vi "Advance Stories.vi"(11 "market":T1) -> (3 "market out":T1)   [LabVIEW 2020, in "Full Featured MCP Server.lvlib"]
doc: "Publishes the story steps that are due. After a step the story takes its good or its bad branch (Good Outcome.vi with the odds of the step and the quality of the lead stock) and the next step is scheduled; a story without a next step ends. Stories that are not due yet wait."
uses:
  Full Featured MCP Server.lvlib
  Market State.ctl
  News Item.ctl
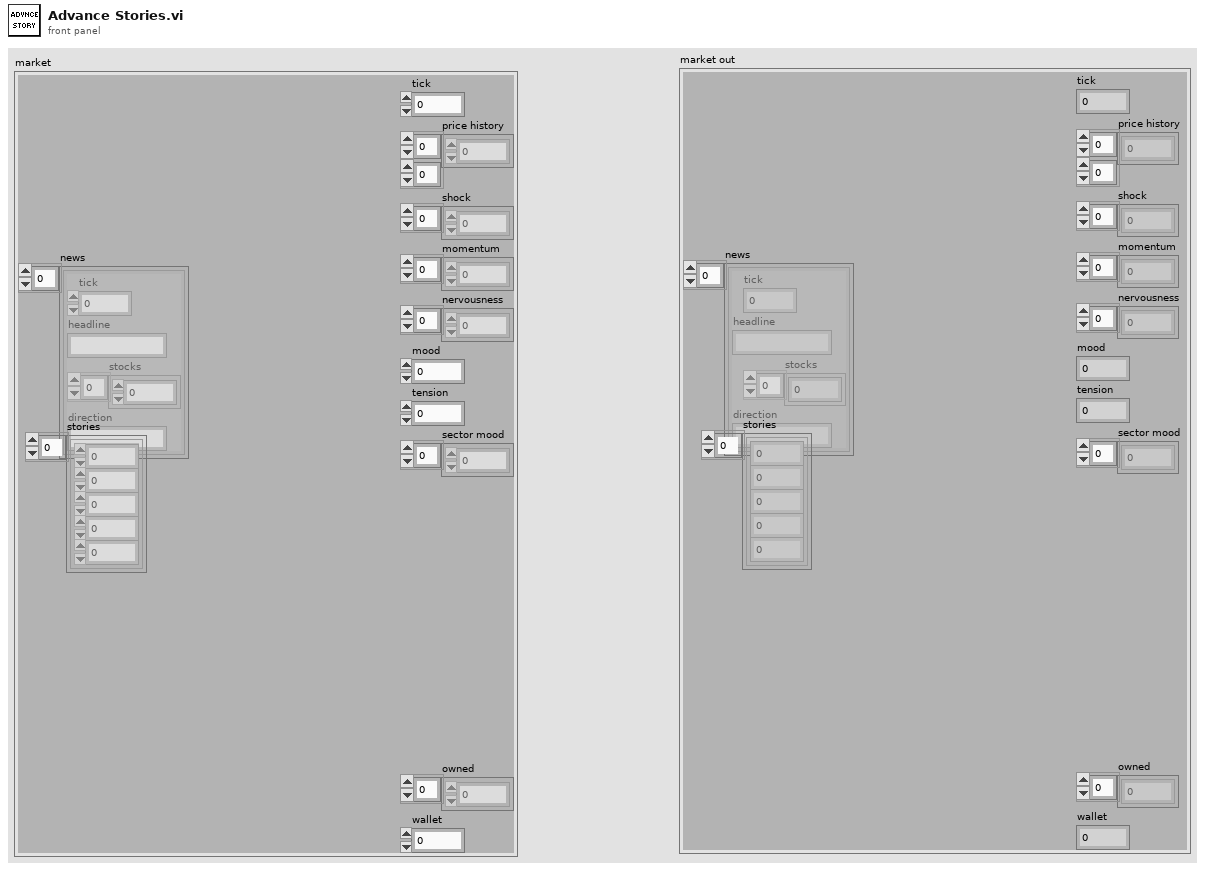
[diagram p1: front panel]
types:
  T1 = typedef "Full Featured MCP Server.lvlib/Market State.ctl" = cluster{"tick":i32, "price history":dbl[][], "shock":dbl[], "momentum":dbl[], "nervousness":dbl[], "mood":dbl, "tension":dbl, "sector mood":dbl[], "news":T2[], "stories":cluster{"arc":i32, "step":i32, "due":i32, "stock":i32, "other":i32}[], "owned":i32[], "wallet":dbl}
  T2 = typedef "Full Featured MCP Server.lvlib/News Item.ctl" = cluster{"tick":i32, "headline":string, "stocks":i32[], "direction":string}
  T3 = cluster{"event":cluster{"headline":string, "scope":enum16{"one stock", "two stocks", "sector", "market"}, "direction":string, "jump":dbl, "follow":dbl, "jump other":dbl, "follow other":dbl}, "delay min":i32, "delay max":i32, "odds":dbl, "next if good":i32, "next if bad":i32}[]
  T4 = cluster{"arc":i32, "step":i32, "due":i32, "stock":i32, "other":i32}[]
  T5 = cluster{"event":cluster{"headline":string, "scope":enum16{"one stock", "two stocks", "sector", "market"}, "direction":string, "jump":dbl, "follow":dbl, "jump other":dbl, "follow other":dbl}, "delay min":i32, "delay max":i32, "odds":dbl, "next if good":i32, "next if bad":i32}
  T6 = cluster{"headline":string, "scope":enum16{"one stock", "two stocks", "sector", "market"}, "direction":string, "jump":dbl, "follow":dbl, "jump other":dbl, "follow other":dbl}
  T7 = cluster{"tick":i32, "price history":dbl[][], "shock":dbl[], "momentum":dbl[], "nervousness":dbl[], "mood":dbl, "tension":dbl, "sector mood":dbl[], "news":cluster{"tick":i32, "headline":string, "stocks":i32[], "direction":string}[], "stories":cluster{"arc":i32, "step":i32, "due":i32, "stock":i32, "other":i32}[], "owned":i32[], "wallet":dbl}
  T8 = cluster{"arc":i32, "step":i32, "due":i32, "stock":i32, "other":i32}
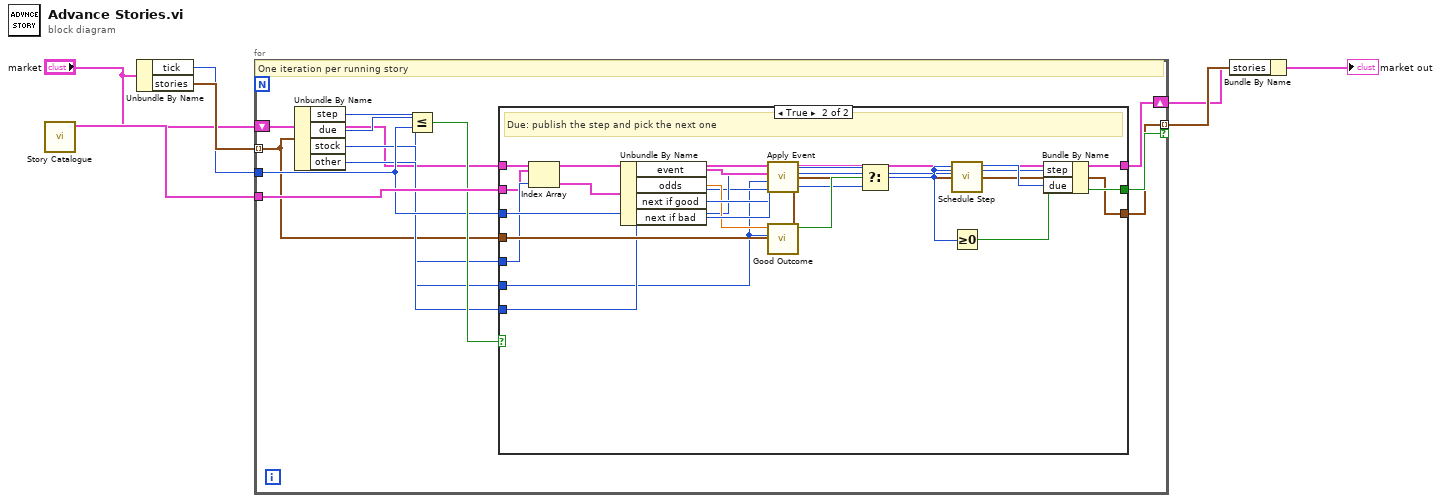
[diagram p0: block diagram]
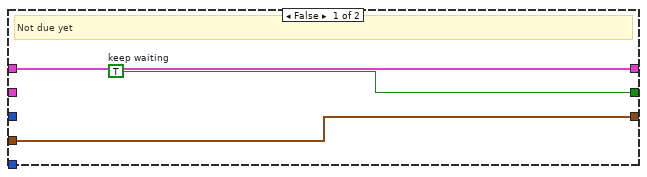
[diagram p2: hidden frame]
diagram:
  n1 = call "Story Catalogue.vi"() -> ("steps"=w4:T3)  [unwired: 10 in, 1 out]
  n2 = Unbundle By Name("market") -> ("tick"=w2:i32, "stories"=w3:T4)
  n3 = for {
    shift-right: [w9] -> w5
    shift-left: "market" -> [w8]
    tunnel: w3 -> [w10] mode=indexing
    tunnel: w2 -> [w15]
    tunnel: w4 -> [w17]
    tunnel: [w18] -> w6 mode=indexing if=w19
    # "One iteration per running story"
    n4 = Unbundle By Name(w10) -> ("step"=w11:i32, "due"=w12:i32, "stock"=w13:i32, "other"=w14:i32)
    n5 = Less Or Equal?(x=w12, y=w15) -> (x <= y?=w16:bool)
    n6 = case shown="True" w16 {
      tunnel: w8 -> [w20 w25]
      tunnel: w17 -> [_ w23]
      tunnel: w15 -> [_ w28]
      tunnel: w10 -> [w21 w29]
      tunnel: w11 -> [_ w24]
      tunnel: w13 -> [_ w26]
      tunnel: w14 -> [_ w27]
      tunnel: [w20 w30] -> w9
      tunnel: [w22 w32] -> w19
      tunnel: [w21 w31] -> w18
      frame False {
        w22 = TRUE  # keep waiting
        # "Not due yet"
      }
      frame True {
        # "Due: publish the step and pick the next one"
        n7 = Index Array(array=w23, index=w24) -> (element=w33:T5)
        n8 = Unbundle By Name(w33) -> ("event"=w34:T6, "odds"=w35:dbl, "next if good"=w36:i32, "next if bad"=w37:i32)
        n9 = call "Apply Event.vi"("other"=w27, "stock"=w26, "event"=w34, "market"=w25) -> ("market out"=w30:T7)  [unwired: 7 in]
        n10 = call "Good Outcome.vi"("stock"=w26, "odds"=w35) -> ("good?"=w38:bool)  [unwired: 9 in]
        n11 = Select(t=w36, s=w38, f=w37) -> (s? t:f=w39:i32)
        n12 = call "Schedule Step.vi"("now"=w28, "step"=w39) -> ("due"=w40:i32)  [unwired: 9 in]
        n13 = Greater Or Equal To 0?(x=w39) -> (x >= 0?=w32:bool)
        n14 = Bundle By Name(cluster=w29, "step"=w39, "due"=w40) -> (w31:T8)
      }
    }
  }
  n15 = Bundle By Name(cluster=w5, "stories"=w6) -> (→"market out":T1)
